vi "AddChannel.vi"(8 "error in (no error)":errorcluster, 10 "Channel":refnum<class "Channel.lvclass">, 11 "object in":refnum<class "ChannelsManager.lvclass">) -> (0 "error out":errorcluster, 3 "object out":refnum<class "ChannelsManager.lvclass">)   [LabVIEW 2021, in "Channel.lvlib" / "ChannelsManager.lvlib" / "ChannelsManager.lvclass"]
doc: "Adds the channel"
uses:
  ChannelsManager.lvclass
  Channel_class/Channel.lvclass
  ChannelsManager.lvclass/ChannelsManager.ctl
  Configuration_class/Configuration.lvclass
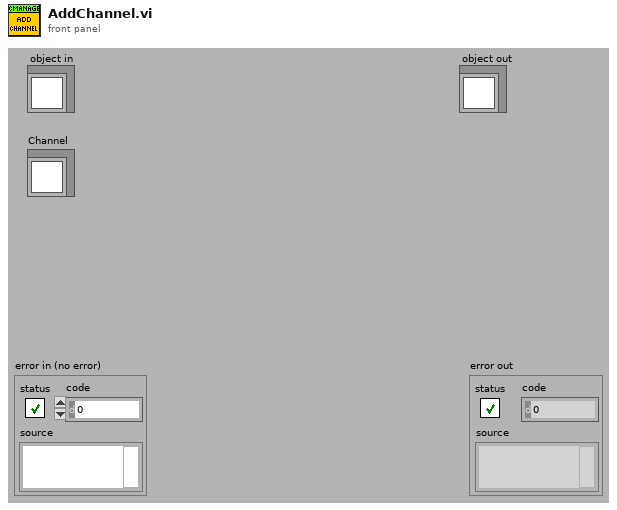
[diagram p1: front panel]
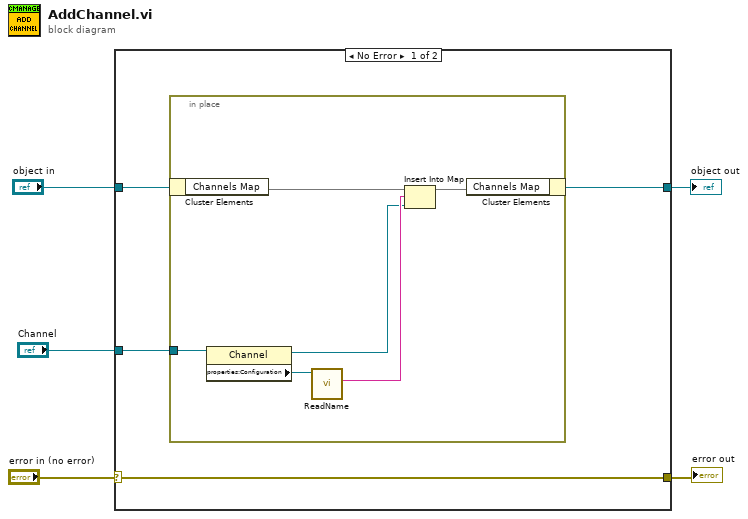
[diagram p0: block diagram]
diagram:
  n1 = case shown="No Error" "error in (no error)" {
    selector: "error in (no error)" -> [w9 w17]
    tunnel: [w9 w17] -> w4
    tunnel: [w7 w16] -> w2
    tunnel: "object in" -> [w8 w16]
    tunnel: "Channel" -> [w6 _]
    frame No Error {
      n2 = in-place {
        in-place-border: w6 -> [w13]
        n3 = in-place-cluster #1(w8) -> ("Channels Map"=w15:map{string, refnum<class "Channel.lvclass">})
        n4 = property class="Channel"(reference=w13) -> (reference out=w10:refnum<class "Channel.lvclass">, "properties:Configuration"=w12:refnum<class "Configuration.lvclass">)  [unwired: 1 in, 1 out]
        n5 = call-dynamic "ReadName.vi"("object in"=w12) -> ("Name"=w11:string)  [unwired: 8 in, 2 out]
        n6 = Insert Into Map(map in=w15, key=w11, value=w10) -> (map out=w14:map{string, refnum<class "Channel.lvclass">})  [unwired: 2 out]
        n7 = in-place-cluster #1("Channels Map"=w14) -> (w7:refnum<class "ChannelsManager.lvclass">)
      }
    }
    frame Error {
    }
  }
  "error out" <- w4
  "object out" <- w2
